vi "INI_Rebuild Property Files.vi"() -> (2 "Why are we here?":T1, 3 "Rebuild Property Files":bool)   [LabVIEW 2023]
doc: "Check to see if LV ini settings indicate scripting or private methods have been turned on since the BundleMagic help files were built."
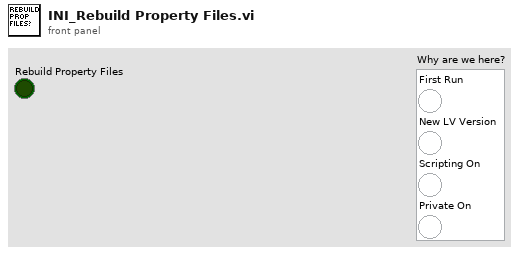
[diagram p1: front panel]
types:
  T1 = cluster{"First Run":bool, "New LV Version":bool, "Scripting On":bool, "Private On":bool}
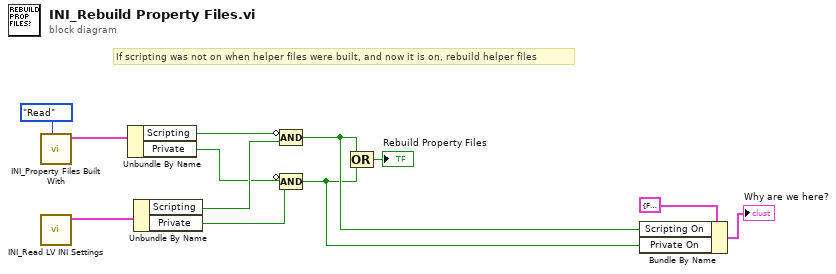
[diagram p0: block diagram]
diagram:
  # "If scripting was not on when helper files were built, and now it is on, rebuild helper files"
  n1 = call "INI_Property Files Built With.vi"("File Action"=enum16{"Read", "Write"}."Read") -> ("Property Files Built With"=w11:cluster{"Scripting":bool, "Private":bool})  [unwired: 10 in]
  n2 = call "INI_Read LV INI Settings.vi"() -> ("LabVIEW INI Settings"=w10:cluster{"Scripting":bool, "Private":bool})  [unwired: 10 in, 1 out]
  n3 = Unbundle By Name(w11) -> ("Scripting"=w9:bool, "Private"=w7:bool)
  n4 = Unbundle By Name(w10) -> ("Scripting"=w8:bool, "Private"=w6:bool)
  n5 = Compound Arithmetic op=AND(invert w9, w8) -> (w2:bool)
  n6 = Compound Arithmetic op=AND(invert w7, w6) -> (w1:bool)
  n7 = Compound Arithmetic op=OR(w2, w1) -> (→"Rebuild Property Files":bool)
  n8 = Bundle By Name(cluster=T1 {"First Run"=FALSE, "New LV Version"=FALSE, "Scripting On"=FALSE, "Private On"=FALSE} ("Why are we here?"), "Scripting On"=w2, "Private On"=w1) -> (→"Why are we here?":T1)
